vi "Initialize.vi"(8 "error in":errorcluster, 10 "parameters":variant, 11 "cRIO in":refnum<class "PLTarget cRIO.lvclass">) -> (0 "error out":errorcluster, 2 "summary":T2[](array[typedef]), 3 "data value reference":T1)   [LabVIEW 2013, in "PLTarget cRIO.lvclass"]
doc: "This Vi initializes the data of a node its default state.\nThe object is not created inside of this ViI, beacuase it is created from a File depending on user selection."
uses:
  PLTarget cRIO.lvclass
  <vilib>/NI/Configuration Framework/Node/Summary.ctl
  <vilib>/NI/Configuration Framework/Node/NodeRef.ctl
  <vilib>/NI/Configuration Framework/Node/NISE_CEF_Node.lvclass
  PLTarget cRIO.lvclass/PLTarget cRIO.ctl
  <vilib>/NI/Tag Bus Module Framework/root configuration/Target Types.ctl
  Framework Configuration Classes/target configuration/PL_Target Configuration.lvclass/PL_Target Configuration.ctl
  Configuration Editor/Classes/Targets/Targets.lvclass
  <vilib>/NI/Tag Bus Module Framework/root configuration/TBM configuration.lvclass
  Framework Configuration Classes/target configuration/PL_Target Configuration.lvclass
  <vilib>/NI/Configuration Framework/serializable configuration/NISE_CEF_serializable configuration.lvclass
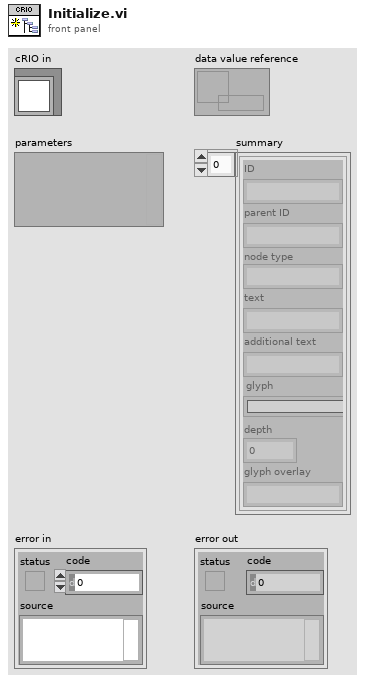
[diagram p1: front panel]
types:
  T1 = typedef "NISE_CEF_Node.lvclass/NodeRef.ctl" = refnum<data-value>
  T2 = typedef "NISE_CEF_Node.lvclass/Summary.ctl" = cluster{"ID":string, "parent ID":string, "node type":string, "text":string, "additional text":string, "glyph":string, "depth":i32, "glyph overlay":string}
  T3 = typedef "TBM configuration.lvclass/Target Types.ctl" = enum16{"Windows", "Mac", "Linux", "Linux RT ARM", "VxWorks", "Pharlap", "Other", "Linux RT x64"}
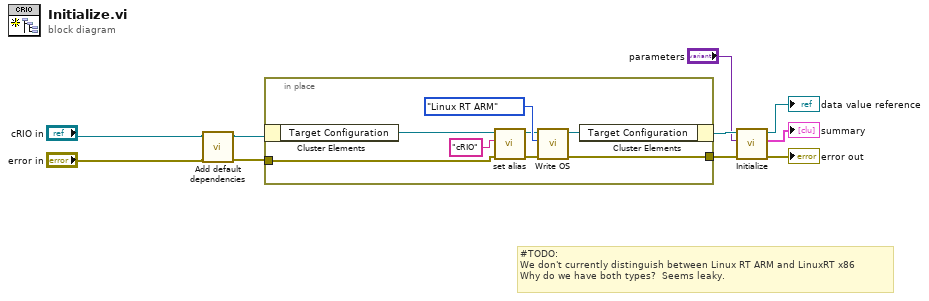
[diagram p0: block diagram]
diagram:
  # "#TODO:\nWe don't currently distinguish between Linux RT ARM and LinuxRT x86\nWhy do we have both types?  Seems leaky."
  n1 = call "Add default dependencies.vi"("error in (no error)"="error in", "Targets in"="cRIO in") -> ("error out"=w3:errorcluster, "Targets out"=w2:refnum<class "PLTarget cRIO.lvclass">)  [unwired: 8 in]
  n2 = in-place {
    in-place-border: [w16] -> w7
    in-place-border: w3 -> [w17]
    n3 = in-place-cluster #1(w2) -> ("Target Configuration"=w11:refnum<class "PL_Target Configuration.lvclass">)
    n4 = call <vilib>:"set alias.vi"("error in"=w17, "alias"="cRIO" ("name"), "configuration in"=w11) -> ("error out"=w13:errorcluster, "configuration out"=w14:refnum<class "PL_Target Configuration.lvclass">)  [unwired: 7 in]
    n5 = call "Write OS.vi"("error in"=w13, "Target Types"=Target_Types."Linux RT ARM" ("OS"), "PL_Target Configuration in"=w14) -> ("error out"=w16:errorcluster, "PL_Target Configuration out"=w12:refnum<class "PL_Target Configuration.lvclass">)  [unwired: 7 in]
    n6 = in-place-cluster #1("Target Configuration"=w12) -> (w6:refnum<class "PLTarget cRIO.lvclass">)
  }
  n7 = call-parent "Initialize.vi"("error in"=w7, "parameters"="parameters", "node in"=w6) -> ("error out"=→"error out":errorcluster, "summary"=→"summary":T2[], "data value reference"=→"data value reference":T1)  [unwired: 6 in]
